vi "setSerializedData.vi"(0 "reference":refnum<class "InterfaceNode.lvclass">, 1 "parent":refnum<class "AbstractNode.lvclass">, 2 "children":refnum<class "AbstractNode.lvclass">[](array[class]), 3 "xmlOut":string, 5 "error in (no error)":errorcluster) -> (14 "reference out":refnum<class "InterfaceNode.lvclass">, 19 "error out":errorcluster)   [LabVIEW 2020, in "InterfaceNode.lvclass"]
doc: "setSerializedData"
uses:
  <resource>/Framework/Providers/Open_GDS/UML/InterfaceNode_class/InterfaceNode.lvclass
  C:/Program Files (x86)/National Instruments/LabVIEW 2020/resource/Framework/Providers/Open_GDS/UML/ClassNode_class/ClassNode.lvclass
  C:/Program Files (x86)/National Instruments/LabVIEW 2020/resource/Framework/Providers/Open_GDS/UML/RectangularNode_class/RectangularNode.lvclass
  C:/Program Files (x86)/National Instruments/LabVIEW 2020/resource/Framework/Providers/Open_GDS/UML/AbstractNode_class/AbstractNode.lvclass
  <resource>/Framework/Providers/Open_GDS/UML/AbstractNode_class/AbstractNode.lvclass
  <resource>/Framework/Providers/Open_GDS/UML/General/Rectangle/Rectangle Rectangle2D.ctl
  <resource>/Framework/Providers/Open_GDS/UML/MultiLineString_class/MultiLineString.lvclass
  <resource>/Framework/Providers/Open_GDS/UML/ClassNode_class/ClassNode.lvclass
  <resource>/Framework/Providers/Open_GDS/UML/RectangularNode_class/RectangularNode.lvclass
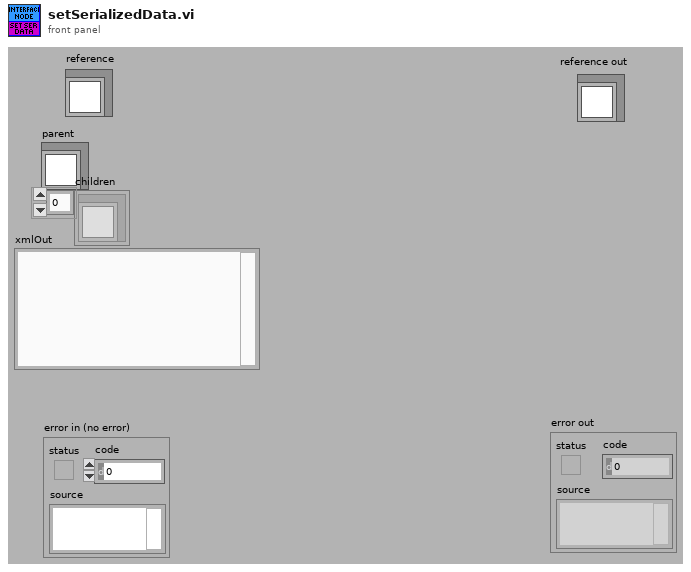
[diagram p1: front panel]
types:
  T1 = typedef "Rectangle Rectangle2D.ctl" = cluster{"x":dbl, "y":dbl, "width":dbl, "height":dbl}
  T2 = cluster{"Base class":cluster{"Base class":cluster{"parent":refnum<k1>, "children":refnum<k1>[], "Hidden":bool}, "bounds":T1}, "midHeight":dbl, "botHeight":dbl, "name":refnum<k1>, "attributes":refnum<k1>, "DEFAULT_COMPARTMENT_HEIGHT":i32, "DEFAULT_WIDTH":i32, "DEFAULT_HEIGHT":i32}
  T3 = cluster{"Base class":cluster{"Base class":cluster{"parent":refnum<k1>, "children":refnum<k1>[], "Hidden":bool}, "bounds":T1}, "midHeight":dbl, "botHeight":dbl, "name":refnum<k1>, "attributes":refnum<k1>, "methods":refnum<k1>, "DEFAULT_COMPARTMENT_HEIGHT":i32, "DEFAULT_WIDTH":i32, "DEFAULT_HEIGHT":i32, "showMethods":bool, "showAttributes":bool, "ClassPath":path}
  T4 = cluster{"Attributes":cluster{"Base class":cluster{"Base class":cluster{"parent":refnum<k1>, "children":refnum<k1>[], "Hidden":bool}, "bounds":T1}, "midHeight":dbl, "botHeight":dbl, "name":refnum<k1>, "attributes":refnum<k1>, "DEFAULT_COMPARTMENT_HEIGHT":i32, "DEFAULT_WIDTH":i32, "DEFAULT_HEIGHT":i32}, string, string}
  T5 = cluster{"Attributes":cluster{"Base class":cluster{"Base class":cluster{"parent":refnum<k1>, "children":refnum<k1>[], "Hidden":bool}, "bounds":T1}, "midHeight":dbl, "botHeight":dbl, "name":refnum<k1>, "attributes":refnum<k1>, "methods":refnum<k1>, "DEFAULT_COMPARTMENT_HEIGHT":i32, "DEFAULT_WIDTH":i32, "DEFAULT_HEIGHT":i32, "showMethods":bool, "showAttributes":bool, "ClassPath":path}, string, string}
  T6 = typedef "ClassNode.lvclass/ObjectAttributes.ctl" = cluster{"midHeight":dbl, "botHeight":dbl, "name":refnum<class "MultiLineString.lvclass">, "attributes":refnum<class "MultiLineString.lvclass">, "methods":refnum<class "MultiLineString.lvclass">, "DEFAULT_COMPARTMENT_HEIGHT":i32, "DEFAULT_WIDTH":i32, "DEFAULT_HEIGHT":i32, "showMethods":bool, "showAttributes":bool, "ClassPath":path}
  T7 = typedef "RectangularNode.lvclass/ObjectAttributes.ctl" = cluster{"bounds":T1}
  T8 = typedef "AbstractNode.lvclass/ObjectAttributes.ctl" = cluster{"parent":refnum<class "AbstractNode.lvclass">, "children":refnum<class "AbstractNode.lvclass">[], "Hidden":bool}
  T9 = cluster{"Base class":cluster{"parent":refnum<k1>, "children":refnum<k1>[], "Hidden":bool}, "bounds":T1}
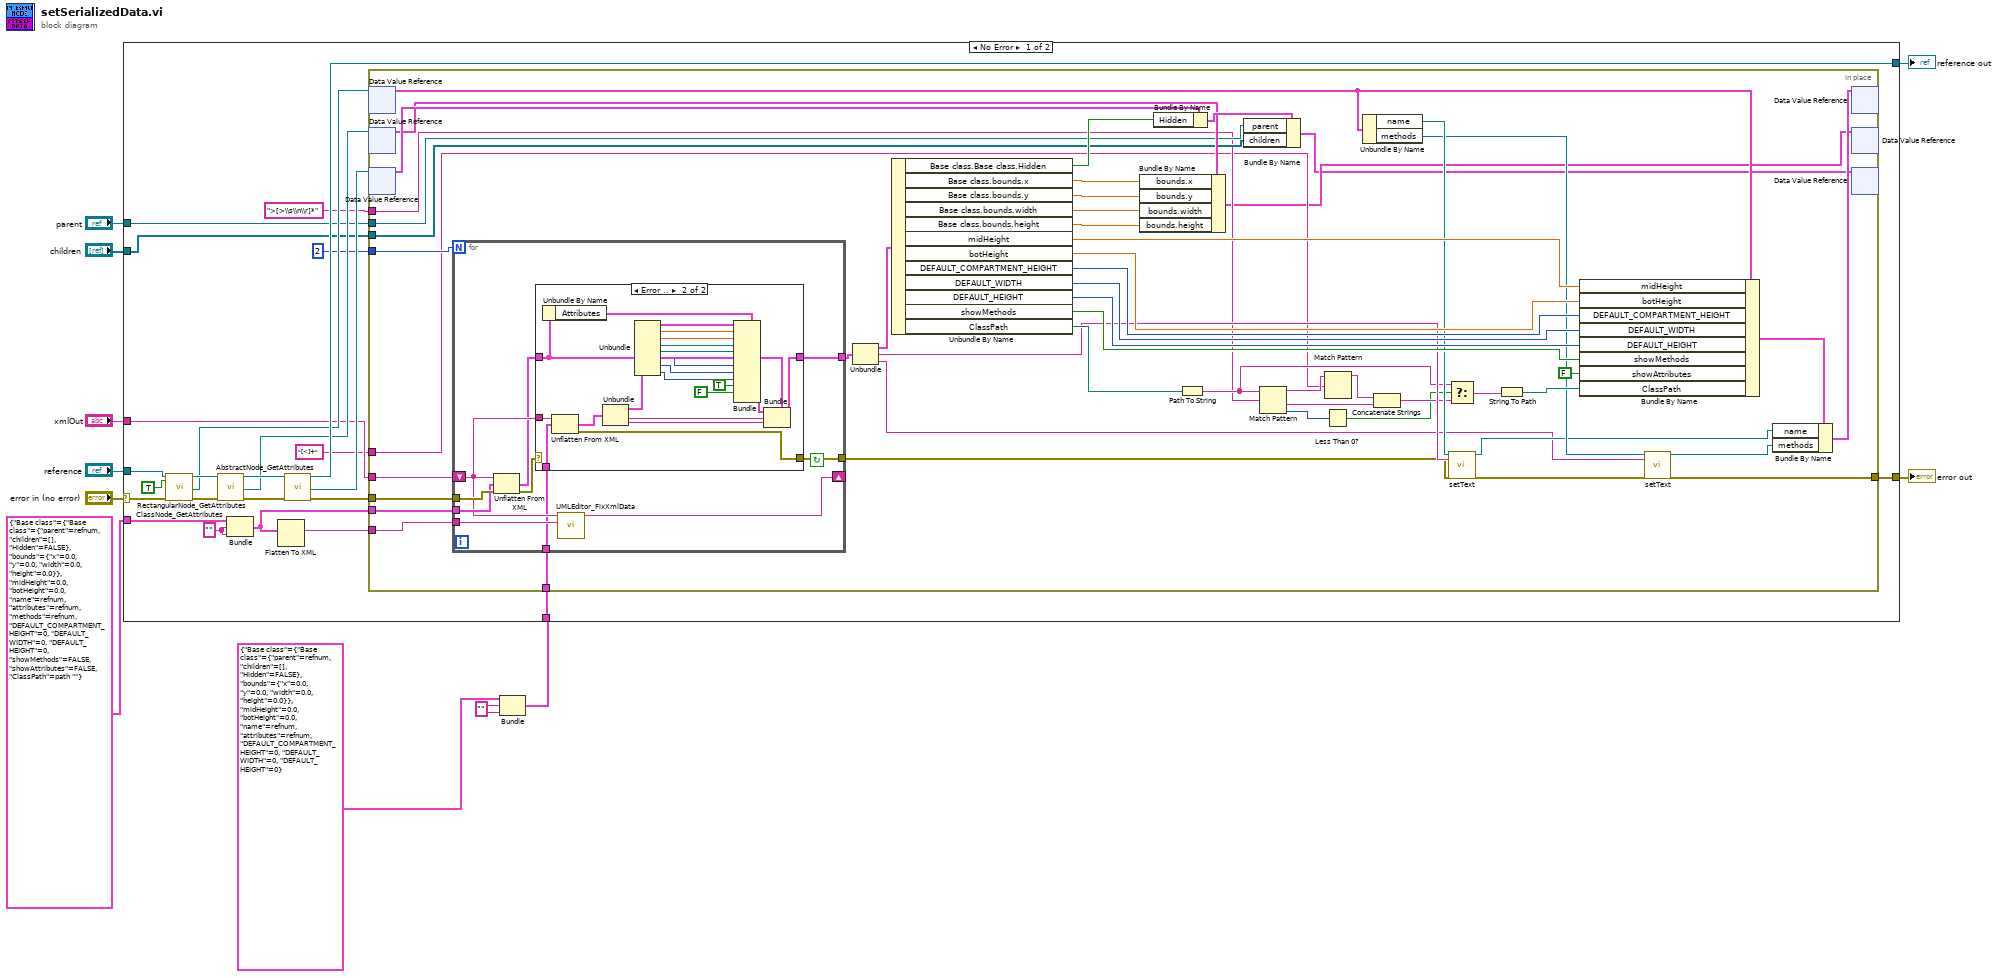
[diagram p0: block diagram]
diagram:
  w3 = ""
  n1 = Bundle("Attributes"=T2 {"Base class"={"Base class"={"parent"=refnum, "children"=[], "Hidden"=FALSE}, "bounds"={"x"=0.0, "y"=0.0, "width"=0.0, "height"=0.0}}, "midHeight"=0.0, "botHeight"=0.0, "name"=refnum, "attributes"=refnum, "DEFAULT_COMPARTMENT_HEIGHT"=0, "DEFAULT_WIDTH"=0, "DEFAULT_HEIGHT"=0}, w3, w3) -> (w1:T4)  [unwired: 1 out]
  n2 = case shown="No Error" "error in (no error)" {
    selector: "error in (no error)" -> [w13 w120]
    tunnel: "reference" -> [w34 w121]
    tunnel: [w33 w120] -> w5
    tunnel: [w35 w121] -> w4
    tunnel: "xmlOut" -> [w19 _]
    tunnel: "parent" -> [w18 _]
    tunnel: "children" -> [w17 _]
    tunnel: T3 {"Base class"={"Base class"={"parent"=refnum, "children"=[], "Hidden"=FALSE}, "bounds"={"x"=0.0, "y"=0.0, "width"=0.0, "height"=0.0}}, "midHeight"=0.0, "botHeight"=0.0, "name"=refnum, "attributes"=refnum, "methods"=refnum, "DEFAULT_COMPARTMENT_HEIGHT"=0, "DEFAULT_WIDTH"=0, "DEFAULT_HEIGHT"=0, "showMethods"=FALSE, "showAttributes"=FALSE, "ClassPath"=path ""} ("Attributes") -> [w31 _]
    tunnel: w1 -> [w14 _]
    frame No Error {
      w32 = ""
      n3 = call <resource>:"ClassNode_GetAttributes.vi"("reference in"=w34, "OnlyGetDvrReference(False)"=TRUE, "error in (no error)"=w13) -> ("reference out"=w29:refnum<class "InterfaceNode.lvclass">, "DataRef"=w25:refnum<data-value>, "error out"=w28:errorcluster)  [unwired: 13 in, 1 out]
      n4 = call <resource>:"RectangularNode_GetAttributes.vi"("reference in"=w29, "error in (no error)"=w28) -> ("reference out"=w27:refnum<class "InterfaceNode.lvclass">, "DataRef"=w24:refnum<data-value>, "error out"=w26:errorcluster)  [unwired: 14 in, 1 out]
      n5 = Bundle("Attributes"=w31, w32, w32) -> (w20:T5)  [unwired: 1 out]
      n6 = Flatten To XML(6:w20) -> (2:w21:string)
      n7 = call <resource>:"AbstractNode_GetAttributes.vi"("reference in"=w27, "error in (no error)"=w26) -> ("reference out"=w35:refnum<class "InterfaceNode.lvclass">, "DataRef"=w23:refnum<data-value>, "error out"=w12:errorcluster)  [unwired: 14 in, 1 out]
      n8 = in-place {
        in-place-border: [w61] -> w33
        in-place-border: 2 -> [w53]
        in-place-border: w12 -> [w52]
        in-place-border: w21 -> [w51]
        in-place-border: w20 -> [w50]
        in-place-border: w19 -> [w49]
        in-place-border: w18 -> [w48]
        in-place-border: w17 -> [w47]
        in-place-border: ">[>\\s\\n\\r]*" ("regular expression") -> [w46]
        in-place-border: "[<]+" ("regular expression") -> [w41]
        in-place-border: w14 -> [w36]
        n9 = in-place-dvr #1(w25) -> (w86:T6)  [unwired: 1 out]
        n10 = in-place-dvr #2(w24) -> (w57:T7)  [unwired: 1 out]
        n11 = in-place-dvr #3(w23) -> (w59:T8)  [unwired: 1 out]
        n12 = for {
          N: w53 -> [_]
          tunnel: w52 -> [w96]
          tunnel: [w87] -> w63
          tunnel: [w88] -> w60
          tunnel: w51 -> [w95]
          tunnel: w50 -> [w94]
          shift-right: [w93] -> _
          shift-left: w49 -> [w91]
          tunnel: w36 -> [w90]
          stop <- w87 continue-if-true
          n13 = Unflatten From XML(xml string=w91, type=w94, error in (no error)=w96) -> (value=w89:T5, error out=w92:errorcluster)
          n14 = case shown="Error .." w92 {
            selector: w92 -> [w97 _]
            tunnel: w91 -> [_ w119]
            tunnel: w90 -> [_ w118]
            tunnel: w89 -> [w98 w111]
            tunnel: [w98 w116] -> w88
            tunnel: [w97 w99] -> w87
            frame No Error {
            }
            frame Error {
              n15 = Unbundle By Name(w111) -> ("Attributes"=w110:T3)
              n16 = Unflatten From XML(xml string=w119, type=w118) -> (value=w117:T4, error out=w99:errorcluster)  [unwired: 1 in]
              n17 = Unbundle(w117) -> ("Attributes"=w113:T2, w114:string, w115:string)
              n18 = Unbundle(w113) -> ("Base class"=w109:T9, "midHeight"=w108:dbl, "botHeight"=w107:dbl, "name"=w106:refnum<k1>, "attributes"=w105:refnum<k1>, "DEFAULT_COMPARTMENT_HEIGHT"=w104:i32, "DEFAULT_WIDTH"=w103:i32, "DEFAULT_HEIGHT"=w102:i32)
              n19 = Bundle(cluster=w110, "Base class"=w109, "midHeight"=w108, "botHeight"=w107, "name"=w106, "attributes"=w105, "DEFAULT_COMPARTMENT_HEIGHT"=w104, "DEFAULT_WIDTH"=w103, "DEFAULT_HEIGHT"=w102, "showMethods"=TRUE, "showAttributes"=FALSE ("showMethods")) -> (w112:T3)  [unwired: 2 in]
              n20 = Bundle(cluster=w111, "Attributes"=w112, w114, w115) -> (w116:T5)
            }
          }
          n21 = call <resource>:"UMLEditor_FixXmlData.vi"("XmlTemplateIn"=w95, "xmlIn"=w91) -> ("XML OUt"=w93:string)  [unwired: 9 in]
        }
        n22 = Unbundle(w60) -> ("Attributes"=w72:T3, w64:string, w37:string)
        n23 = Unbundle By Name(w72) -> ("Base class.Base class.Hidden"=w71:bool, "Base class.bounds.x"=w70:dbl, "Base class.bounds.y"=w69:dbl, "Base class.bounds.width"=w68:dbl, "Base class.bounds.height"=w67:dbl, "midHeight"=w85:dbl, "botHeight"=w84:dbl, "DEFAULT_COMPARTMENT_HEIGHT"=w83:i32, "DEFAULT_WIDTH"=w82:i32, "DEFAULT_HEIGHT"=w81:i32, "showMethods"=w80:bool, "ClassPath"=w66:path)
        n24 = Bundle By Name(cluster=w57, "bounds.x"=w70, "bounds.y"=w69, "bounds.width"=w68, "bounds.height"=w67) -> (w40:T7)
        n25 = Bundle By Name(cluster=w59, "Hidden"=w71) -> (w58:T8)
        n26 = Path To String(path=w66) -> (string=w56:string)
        n27 = Bundle By Name(cluster=w58, "parent"=w48, "children"=w47) -> (w39:T8)
        n28 = Match Pattern(string=w56, regular expression=w46) -> (before substring=w45:string, after substring=w44:string, offset past match=w43:i32)  [unwired: 2 out]
        n29 = Less Than 0?(x=w43) -> (x < 0?=w54:bool)
        n30 = Match Pattern(string=w45, regular expression=w41) -> (before substring=w42:string)  [unwired: 4 out]
        n31 = Unbundle By Name(w86) -> ("name"=w77:refnum<class "MultiLineString.lvclass">, "methods"=w76:refnum<class "MultiLineString.lvclass">)
        n32 = Concatenate Strings(w42, w44) -> (w55:string)
        n33 = Select(t=w56, s=w54, f=w55) -> (s? t:f=w65:string)
        n34 = call-dynamic "setText.vi"("reference"=w77, "text"=w64, "error in (no error)"=w63) -> ("reference out"=w75:refnum<class "MultiLineString.lvclass">, "error out"=w62:errorcluster)  [unwired: 15 out]
        n35 = String To Path(string=w65) -> (path=w79:path)
        n36 = Bundle By Name(cluster=w86, "midHeight"=w85, "botHeight"=w84, "DEFAULT_COMPARTMENT_HEIGHT"=w83, "DEFAULT_WIDTH"=w82, "DEFAULT_HEIGHT"=w81, "showMethods"=w80, "showAttributes"=FALSE, "ClassPath"=w79) -> (w78:T6)
        n37 = call-dynamic "setText.vi"("reference"=w76, "text"=w37, "error in (no error)"=w62) -> ("reference out"=w74:refnum<class "MultiLineString.lvclass">, "error out"=w61:errorcluster)  [unwired: 15 out]
        n38 = Bundle By Name(cluster=w78, "name"=w75, "methods"=w74) -> (w73:T6)
        n39 = in-place-dvr #1(w73) -> ()  [unwired: 2 out]
        n40 = in-place-dvr #2(w40) -> ()  [unwired: 2 out]
        n41 = in-place-dvr #3(w39) -> ()  [unwired: 2 out]
      }
    }
    frame Error {
    }
  }
  "reference out" <- w4
  "error out" <- w5
